vi "IDs to Names.vi"(10 "IDs":T1) -> (2 "Names":string[](array[string]), 3 "IDs":string[](array[string]))   [LabVIEW 2019, in "Tool Data.lvclass"]
uses:
  Tool Data.lvclass
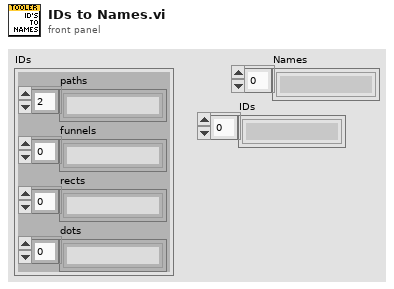
[diagram p1: front panel]
types:
  T1 = cluster{"paths":string[], "funnels":string[], "rects":string[], "dots":string[]}
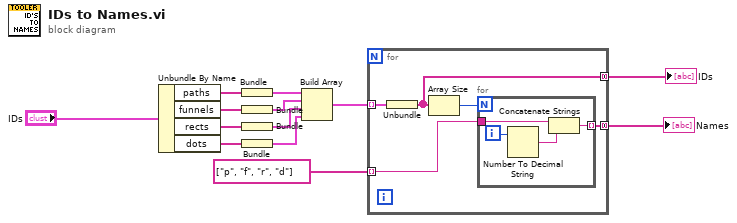
[diagram p0: block diagram]
diagram:
  n1 = Unbundle By Name("IDs") -> ("paths"=w12:string[], "funnels"=w11:string[], "rects"=w10:string[], "dots"=w9:string[])
  n2 = Bundle("paths"=w12) -> (w8:cluster{"paths":string[]})  [unwired: 1 in]
  n3 = Bundle("funnels"=w11) -> (w7:cluster{"funnels":string[]})  [unwired: 1 in]
  n4 = Bundle("rects"=w10) -> (w6:cluster{"rects":string[]})  [unwired: 1 in]
  n5 = Bundle("dots"=w9) -> (w5:cluster{"dots":string[]})  [unwired: 1 in]
  n6 = Build Array(w8, w7, w6, w5) -> (w3:cluster{"dots":string[]}[])
  n7 = for {
    tunnel: string[] ["p", "f", "r", "d"] -> [w16] mode=indexing
    tunnel: w3 -> [w18] mode=indexing
    tunnel: [w15] -> w2 mode=concatenating
    tunnel: [w14] -> w1 mode=concatenating
    n8 = Unbundle(w18) -> ("dots"=w14:string[])
    n9 = Array Size(array=w14) -> (size(s)=w17:i32)
    n10 = for {
      N: w17 -> [_]
      tunnel: w16 -> [w21]
      tunnel: [w19] -> w15 mode=indexing
      i -> [w22]
      n11 = Number To Decimal String(number=w22) -> (decimal integer string=w20:string)  [unwired: 1 in]
      n12 = Concatenate Strings(w21, w20) -> (w19:string)
    }
  }
  "Names" <- w2
  "IDs" <- w1
